vi "create event from run.vi"(7 "Time Stamp (now)":timestamp format="%<%x %.3X>T", 9 "Type":enum16{"INFO", "FLAG", "ERROR", "SUCCESS"}(ring), 10 "Name":string, 11 "run":refnum<class "Run.lvclass">) -> (0 "error out":errorcluster, 3 "event":refnum<class "event.lvclass">)   [LabVIEW 2020, in "nominal core steps.lvlib"]
doc: "Creates an event which flags a time range in Nominal."
uses:
  nominal core steps.lvlib
  <vilib>/Nominal/Nominal IO Client/lv_src/Run/Run.lvclass
  <vilib>/Nominal/Nominal IO Client/lv_src/event/event.lvclass
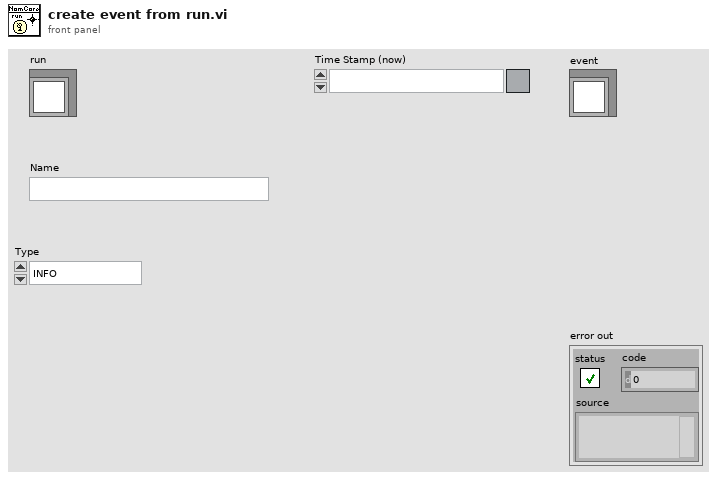
[diagram p1: front panel]
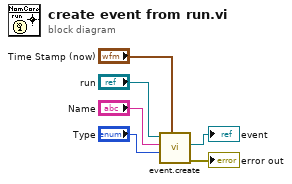
[diagram p0: block diagram]
diagram:
  n1 = call <vilib>:"event.create.vi"("Time Stamp (now)"="Time Stamp (now)", "Type"="Type", "Name"="Name", "Run in"="run") -> ("error out"=→"error out":errorcluster, "event"=→"event":refnum<class "event.lvclass">)  [unwired: 5 in, 1 out]
